vi "Load Scale Parameter.vi"(7 "section":string="Motor", 8 "error in (no error)":errorcluster, 9 "Offset Key":string="Speed_In_Offset", 10 "Gain Key":string="Speed_In_Gain", 11 "config file in":path) -> (0 "error out":errorcluster, 2 "Scale Parameters":cluster{"Gain":dbl, "Offset":dbl}, 3 "config file out":path)   [LabVIEW 2021]
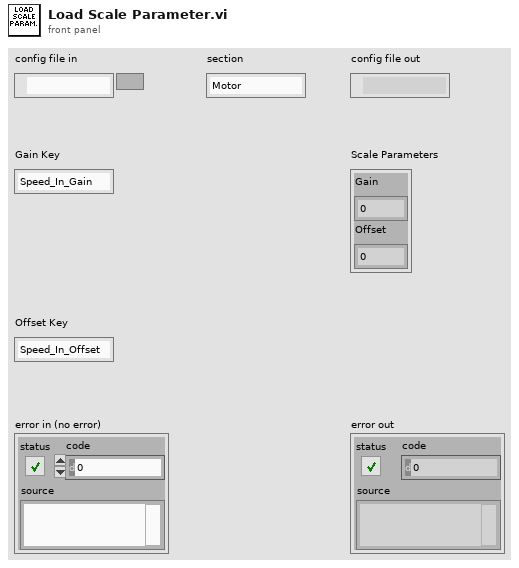
[diagram p1: front panel]
types:
  T1 = cluster{"default value 1":dbl, "default value 1":dbl}
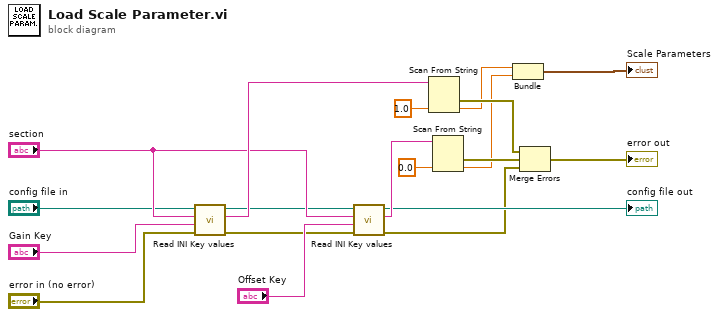
[diagram p0: block diagram]
diagram:
  n1 = call "Read INI Key values.vi"("error in (no error)"="error in (no error)", "key"="Gain Key", "section"="section", "Path In"="config file in") -> ("error out"=w8:errorcluster, "value"=w10:string, "Path Out"=w6:path)  [unwired: 5 in]
  n2 = call "Read INI Key values.vi"("error in (no error)"=w8, "key"="Offset Key", "section"="section", "Path In"=w6) -> ("error out"=w1:errorcluster, "value"=w14:string, "Path Out"=→"config file out":path)  [unwired: 5 in]
  n3 = Scan From String(input string=w10, default 1=1.0 ("default value 1")) -> (error out=w17:errorcluster, output 1=w12:dbl)  [unwired: 3 in, 2 out]
  n4 = Scan From String(input string=w14, default 1=0.0 ("default value 1")) -> (error out=w18:errorcluster, output 1=w15:dbl)  [unwired: 3 in, 2 out]
  n5 = Bundle("default value 1"=w12, "default value 1"=w15) -> (→"Scale Parameters":T1)  [unwired: 1 in]
  n6 = Merge Errors(w17, w18, w1) -> (→"error out":errorcluster)
